vi "[ex ce] CalcExpress & LabVIEW speed.vi"() -> ()   [LabVIEW 2021]
doc: "<B>Run speed example</B>\n\nThis example compares speed of CalcExpress and LabVIEW functions for formula evaluation.\n\n::: CalcExpress Toolkit :::\nCopyright (c) 2000-2026 Konstantin Shifershteyn. All rights reserved."
uses:
  <vilib>/gmath/NI_Gmath.lvlib
panel:
  out "LV error":errorcluster
  out "CE error":errorcluster
  in  "use":T1(ring)=enum."LV formula parser"
  in  "stop":bool
  out "graph2":cluster{dbl[], dbl[]}(graph)
  in  "formula":string="x = sin(i+w) * cos(i/4);\ny = cos(i/2) * sin(i);"
  out "Time CE":u32 caption="calc time, ms"
  out "graph1":cluster{dbl[], dbl[]}(graph)
  out "Time LV":u32 caption="calc time, ms"
  in  "N points":i32=10000
  # "LabVIEW functions"
  # "CalcExpress"
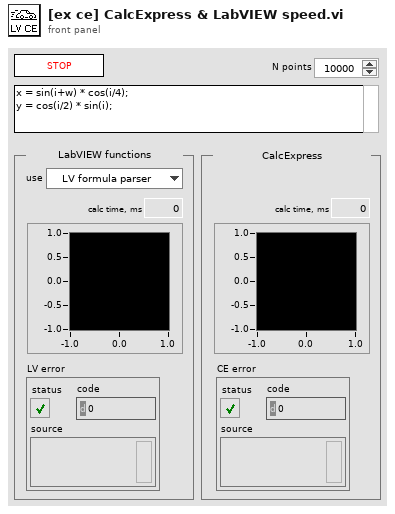
[diagram p1: front panel]
types:
  T1 = enum16{"LV functions", "LV formula node", "LV formula parser"}
  T2 = typedef "VarMan Variable Context Handle.ctl" = i32
  T3 = enum16{"create", "destroy", "set value", "get value"}
  T4 = cluster{"Y Values":dbl[][], "Tables":i32[][][], "Variables input decode":i32[], "Variables output decode":i32[]}
  T5 = cluster{"Output Values":dbl[], "Output Values":dbl[]}
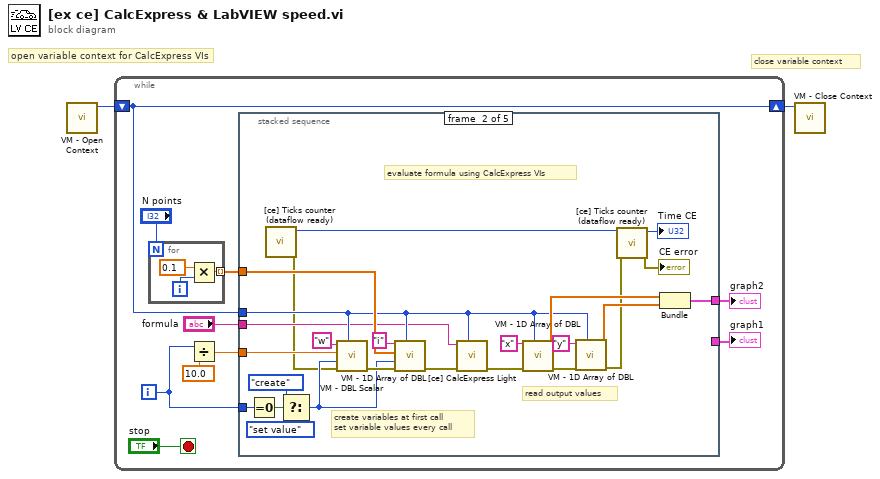
[diagram p0: block diagram]
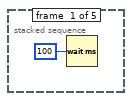
[diagram p2: hidden frame]
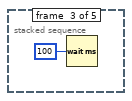
[diagram p3: hidden frame]
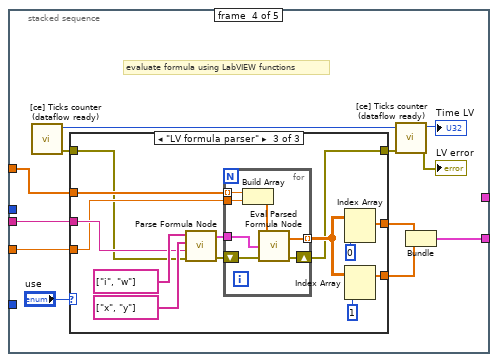
[diagram p4: hidden frame]
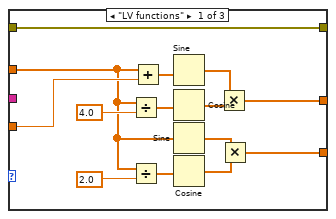
[diagram p5: hidden frame]
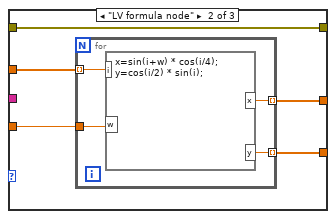
[diagram p6: hidden frame]
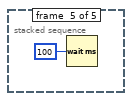
[diagram p7: hidden frame]
diagram:
  # "close variable context"
  # "open variable context for CalcExpress VIs"
  n1 = call "VM - Open Context.vi"() -> ("VC Handle out"=w1:T2)  [unwired: 9 in, 2 out]
  n2 = while {
    shift-left: w1 -> [w10]
    shift-right: [w10] -> w2
    i -> [w5]
    stop <- "stop" stop-if-true
    n3 = for {
      N: "N points" -> [_]
      tunnel: [w13] -> w12 mode=indexing
      i -> [w15]
      n4 = Multiply(x=0.1, y=w15) -> (x*y=w13:dbl)
    }
    n5 = Divide(x=w5, y=10.0) -> (x/y=w8:dbl)
    n6 = stacked-sequence "Sequence" {
      tunnel: w12 -> [_ w37 _ w54 _]
      tunnel: w10 -> [_ w28 _ _ _]
      tunnel: w8 -> [_ w34 _ w51 _]
      tunnel: [_ w33 _ _ _] -> w7
      tunnel: [_ _ _ w50 _] -> w6
      tunnel: w5 -> [_ w23 _ _ _]
      tunnel: "formula" -> [_ w22 _ w48 _]
      frame #0 {
        n7 = Wait (ms)(milliseconds to wait=u32 100) -> ()  [unwired: 1 out]
      }
      frame #1 {
        # "read output values"
        # "create variables at first call\nset variable values every call"
        # "evaluate formula using CalcExpress VIs"
        n8 = Equal To 0?(x=w23) -> (x = 0?=w24:bool)
        n9 = call "[ce] Ticks counter (dataflow ready).vi"() -> ("error out"=w21:errorcluster, "ticks (current-input)"=w20:u32)  [unwired: 5 in, 3 out]
        n10 = Select(t=T3."create", s=w24, f=T3."set value" ("cmd")) -> (s? t:f=w25:T3)
        n11 = call "VM - DBL Scalar.vi"("VC Handle"=w28, "error in"=w21, "cmd"=w25, "value in"=w34, "name_spec"="w" ("name")) -> ("error out"=w36:errorcluster)  [unwired: 1 in, 5 out]
        n12 = call "VM - 1D Array of DBL.vi"("VC Handle"=w28, "error in"=w36, "cmd"=w25, "value in"=w37, "name_spec"="i") -> ("error out"=w38:errorcluster)  [unwired: 1 in, 5 out]
        n13 = call "[ce] CalcExpress Light.vi"("VC Handle"=w28, "error in"=w38, "expression"=w22) -> ("error out"=w30:errorcluster)  [unwired: 6 in, 2 out]
        n14 = call "VM - 1D Array of DBL.vi"("VC Handle"=w28, "error in"=w30, "name_spec"="x" ("var name")) -> ("error out"=w29:errorcluster, "value out"=w41:dbl[])  [unwired: 3 in, 4 out]
        n15 = call "VM - 1D Array of DBL.vi"("VC Handle"=w28, "error in"=w29, "name_spec"="y" ("var name")) -> ("error out"=w19:errorcluster, "value out"=w40:dbl[])  [unwired: 3 in, 4 out]
        n16 = call "[ce] Ticks counter (dataflow ready).vi"("error in"=w19, "ticks in"=w20) -> ("error out"=→"CE error":errorcluster, "ticks (current-input)"=→"Time CE":u32)  [unwired: 3 in, 3 out]
        n17 = Bundle("value out"=w41, "value out"=w40) -> (w33:cluster{"value out":dbl[], "value out":dbl[]})  [unwired: 1 in]
      }
      frame #2 {
        n18 = Wait (ms)(milliseconds to wait=u32 100) -> ()  [unwired: 1 out]
      }
      frame #3 {
        # "evaluate formula using LabVIEW functions"
        n19 = call "[ce] Ticks counter (dataflow ready).vi"() -> ("error out"=w47:errorcluster, "ticks (current-input)"=w46:u32)  [unwired: 5 in, 3 out]
        n20 = case shown="\"LV formula parser\"" "use" {
          tunnel: [w66 w70 w85] -> w53
          tunnel: [w62 w71 w84] -> w52
          tunnel: w51 -> [w58 w72 w79]
          tunnel: w54 -> [w56 w73 w80]
          tunnel: w47 -> [w55 w69 w78]
          tunnel: [w55 w69 w81] -> w45
          tunnel: w48 -> [_ _ w82]
          frame "LV functions" {
            n21 = Divide(x=w56, y=4.0) -> (x/y=w61:dbl[])
            n22 = Divide(x=w56, y=2.0) -> (x/y=w59:dbl[])
            n23 = Add(x=w56, y=w58) -> (x+y=w57:dbl[])
            n24 = Sine(x=w57) -> (sin(x)=w68:dbl[])
            n25 = Cosine(x=w61) -> (cos(x)=w67:dbl[])
            n26 = Sine(x=w56) -> (sin(x)=w64:dbl[])
            n27 = Cosine(x=w59) -> (cos(x)=w63:dbl[])
            n28 = Multiply(x=w68, y=w67) -> (x*y=w66:dbl[])
            n29 = Multiply(x=w64, y=w63) -> (x*y=w62:dbl[])
          }
          frame "LV formula node" {
            n30 = for {
              tunnel: w73 -> [w77] mode=indexing
              tunnel: w72 -> [w76]
              tunnel: [w75] -> w71 mode=indexing
              tunnel: [w74] -> w70 mode=indexing
              n31 = formula code="x=sin(i+w) * cos(i/4);\ny=cos(i/2) * sin(i);"("i"=w77, "w"=w76) -> ("y"=w75:dbl, "x"=w74:dbl)
            }
          }
          frame "LV formula parser" {
            n32 = call <vilib>:"Parse Formula Node.vi"("error in (no error)"=w78, "formula"=w82, "Variables Output"=string[] ["x", "y"], "Variables Input"=string[] ["i", "w"]) -> ("error out"=w91:errorcluster, "Parsed Formula Node"=w90:T4)
            n33 = for {
              shift-right: [w98] -> w81
              shift-left: w91 -> [w97]
              tunnel: w90 -> [w96]
              tunnel: [w95] -> w83 mode=indexing
              tunnel: w80 -> [w94] mode=indexing
              tunnel: w79 -> [w92]
              n34 = Build Array(w94, w92) -> (w93:dbl[])
              n35 = call <vilib>:"Eval Parsed Formula Node.vi"("error in (no error)"=w97, "Parsed Formula Node"=w96, "Input Values"=w93) -> ("error out"=w98:errorcluster, "Output Values"=w95:dbl[])
            }
            n36 = Index Array(array=w83, index (col)=0) -> (element=w85:dbl[])  [unwired: 1 in]
            n37 = Index Array(array=w83, index (col)=1) -> (element=w84:dbl[])  [unwired: 1 in]
          }
        }
        n38 = call "[ce] Ticks counter (dataflow ready).vi"("error in"=w45, "ticks in"=w46) -> ("error out"=→"LV error":errorcluster, "ticks (current-input)"=→"Time LV":u32)  [unwired: 3 in, 3 out]
        n39 = Bundle("Output Values"=w53, "Output Values"=w52) -> (w50:T5)  [unwired: 1 in]
      }
      frame #4 {
        n40 = Wait (ms)(milliseconds to wait=u32 100) -> ()  [unwired: 1 out]
      }
    }
    "graph2" <- w7
    "graph1" <- w6
  }
  n41 = call "VM - Close Context.vi"("VC Handle"=w2) -> ()  [unwired: 9 in, 2 out]
